vi "populate db with default.vi"(0 "SQLite Connection in":refnum<class "Connection.lvclass">, 5 "Input Map":T1[](array[typedef]), 7 "Output Map":T1[](array[typedef]), 9 "table name":string, 11 "error in":errorcluster) -> (4 "SQLite Connection out":refnum<class "Connection.lvclass">, 15 "error out":errorcluster)   [LabVIEW 2014, in "SQLite runtime.lvclass"]
uses:
  SQLite runtime.lvclass
  <vilib>/drjdpowell/SQLite Library/SQL Connection/Connection.lvclass
  <vilib>/NI/Tag Bus/table/data table.ctl
  data map.ctl
  <vilib>/NI/Tag Bus/tag/Data Type.ctl
  sqlite type.ctl
  <vilib>/drjdpowell/SQLite Library/SQL Statement/SQL Statement.lvclass/SQL Statement.ctl
  <vilib>/drjdpowell/SQLite Library/SQL Statement/Bind Text.vi
  <vilib>/drjdpowell/SQLite Library/SQL Statement/Step.vi
  <vilib>/drjdpowell/SQLite Library/SQL Statement/Error Message.vi
  <vilib>/drjdpowell/SQLite Library/SQL Statement/SQL Statement.lvclass
  <vilib>/NI/Tag Bus/table/data table.lvlib
  <vilib>/NI/Tag Bus/tag/tag descriptor.lvclass
panel:
  in  "data table":T4
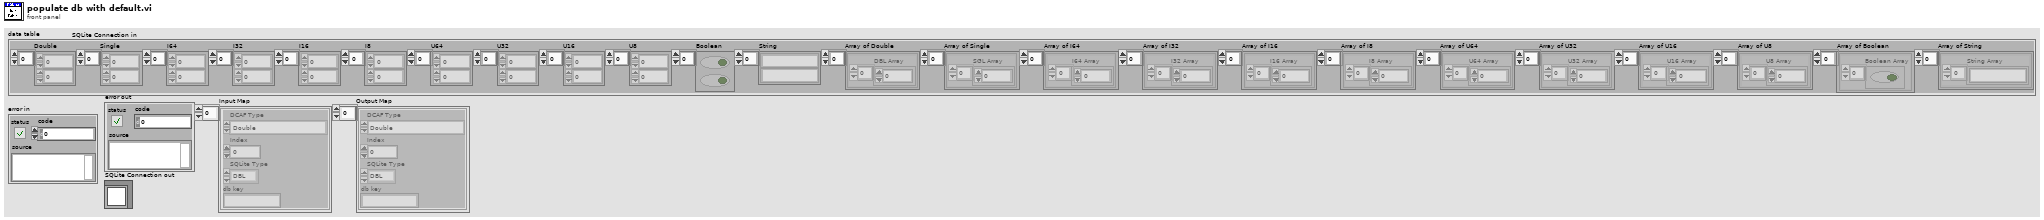
[diagram p1: front panel]
types:
  T1 = typedef "SQLite runtime.lvclass/data map.ctl" = cluster{"DCAF Type":T2, "Index":i32, "SQLite Type":T3, "db key":string}
  T2 = typedef "tag bus.lvlib/tag descriptor.lvclass/Data Type.ctl" = enum16{"Double", "Single", "I64", "I32", "I16", "I8", "U64", "U32", "U16", "U8", "Boolean", "String", "Array of Double", "Array of Single", "Array of I64", "Array of I32", "Array of I16", "Array of I8", "Array of U64", "Array of U32", "Array of U16", "Array of U8", "Array of Boolean", "Array of String"}
  T3 = typedef "SQLite runtime.lvclass/sqlite type.ctl" = enum16{"DBL", "I64", "String"}
  T4 = typedef "tag bus.lvlib/data table.lvlib/data table.ctl" = cluster{"Double":dbl[], "Single":sgl[], "I64":i64[], "I32":i32[], "I16":i16[], "I8":i8[], "U64":u64[], "U32":u32[], "U16":u16[], "U8":u8[], "Boolean":bool[], "String":string[], "Array of Double":cluster{"DBL Array":dbl[]}[], "Array of Single":cluster{"SGL Array":sgl[]}[], "Array of I64":cluster{"I64 Array":i64[]}[], "Array of I32":cluster{"I32 Array":i32[]}[], "Array of I16":cluster{"I16 Array":i16[]}[], "Array of I8":cluster{"I8 Array":i8[]}[], "Array of U64":cluster{"U64 Array":u64[]}[], "Array of U32":cluster{"U32 Array":u32[]}[], "Array of U16":cluster{"U16 Array":u16[]}[], "Array of U8":cluster{"U8 Array":u8[]}[], "Array of Boolean":cluster{"Boolean Array":bool[]}[], "Array of String":cluster{"String Array":string[]}[]}
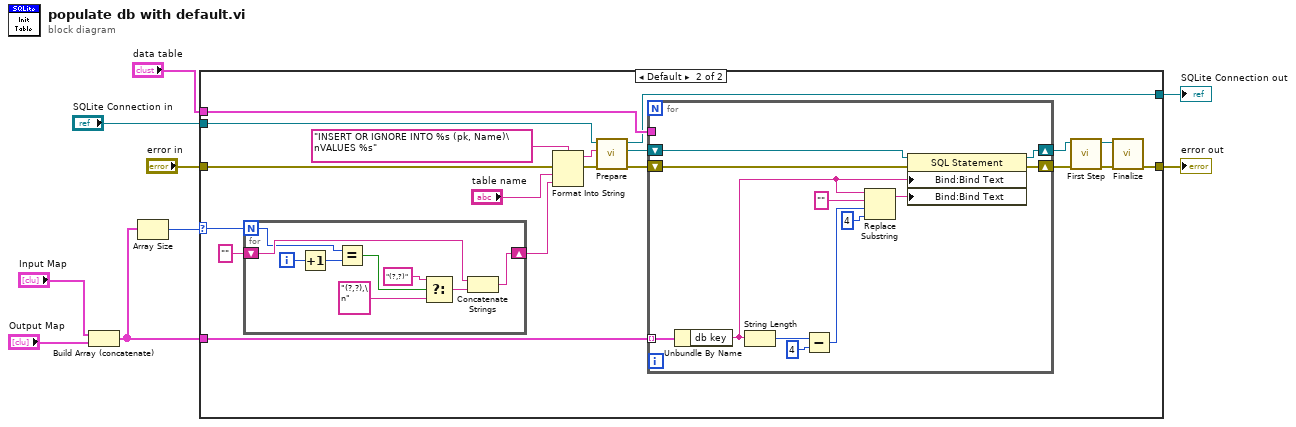
[diagram p0: block diagram]
diagram:
  n1 = Build Array (concatenate)("Input Map", "Output Map") -> (w1:T1[])
  n2 = Array Size(array=w1) -> (size(s)=w9:i32)
  n3 = case shown="Default" w9 {
    selector: w9 -> [_ w30]
    tunnel: "SQLite Connection in" -> [w10 w26]
    tunnel: "data table" -> [_ w17]
    tunnel: w1 -> [_ w20]
    tunnel: [w11 w14] -> w6
    tunnel: "error in" -> [w11 w13]
    tunnel: [w10 w12] -> w4
    frame 0 {
    }
    frame Default {
      n4 = for {
        N: w30 -> [w48]
        shift-right: [w51] -> w27
        shift-left: "" -> [w50]
        i -> [w49]
        n5 = Increment(x=w49) -> (x+1=w43:i32)
        n6 = Equal?(x=w48, y=w43) -> (x = y?=w47:bool)
        n7 = Select(t="(?,?)" ("string"), s=w47, f="(?,?),\n" ("string")) -> (s? t:f=w44:string)
        n8 = Concatenate Strings(w50, w44) -> (w51:string)
      }
      n9 = Format Into String(format string="INSERT OR IGNORE INTO %s (pk, Name)\nVALUES %s" ("delimiter (Tab)"), error in=w13, "table name", w27) -> (resulting string=w24:string, error out=w18:errorcluster)  [unwired: 1 in]
      n10 = call <vilib>:"Prepare.vi"("error in (no error)"=w18, "SQL"=w24, "SQLite Connection in"=w26) -> ("error out"=w19:errorcluster, "SQL Statement out"=w21:refnum<class "SQL Statement.lvclass">, "SQLite Connection out"=w12:refnum<class "Connection.lvclass">)  [unwired: 4 in, 2 out]
      n11 = for {
        shift-right: [w32] -> w23
        shift-left: w21 -> [w42]
        tunnel: w20 -> [w35] mode=indexing
        shift-right: [w31] -> w16
        shift-left: w19 -> [w41]
        tunnel: w17 -> [_]
        n12 = Unbundle By Name(w35) -> ("db key"=w33:string)
        n13 = String Length(string=w33) -> (length=w40:i32)
        n14 = Subtract(x=w40, y=4) -> (x-y=w38:i32)
        n15 = Replace Substring(2:4 ("length (len. of substring)"), 3:w38, 4:"" ("substring (\"\")"), 5:w33) -> (1:w34:string)  [unwired: 1 out]
        n16 = property class="SQL Statement"(reference=w42, error in=w41, "Bind:Bind Text"=w33, "Bind:Bind Text"=w34) -> (reference out=w32:refnum<class "SQL Statement.lvclass">, error out=w31:errorcluster)
      }
      n17 = call <vilib>:"First Step.vi"("error in (no error)"=w16, "SQL Statement in"=w23) -> ("error out"=w15:errorcluster, "SQL Statement out"=w22:refnum<class "SQL Statement.lvclass">)  [unwired: 7 in, 1 out]
      n18 = call <vilib>:"Finalize.vi"("error in (no error)"=w15, "SQL Statement in"=w22) -> ("error out"=w14:errorcluster)  [unwired: 9 in]
    }
  }
  "error out" <- w6
  "SQLite Connection out" <- w4
